vi "Log.vi"(8 "error in":errorcluster, 10 "Log Entry":T1 {"Time" format="%<%x %.3X>T"}, 11 "ILogger in":refnum<class "ILogger.lvclass">) -> (0 "error out":errorcluster, 3 "ILogger out":refnum<class "ILogger.lvclass">)   [LabVIEW 2026, in "ILogger.lvlib" / "ILogger.lvclass"]
doc: "Log the provided entry."
uses:
  ILogger.lvclass
  Type Definitions/Log Entry--cluster.ctl
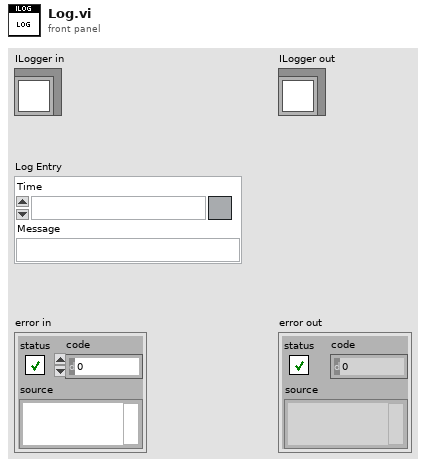
[diagram p1: front panel]
types:
  T1 = typedef "Log Entry--cluster.ctl" = cluster{"Time":timestamp, "Message":string}
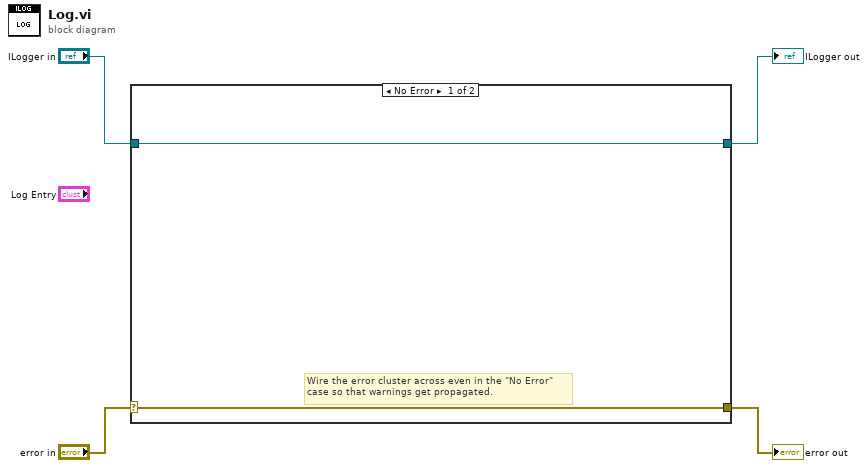
[diagram p0: block diagram]
diagram:
  n1 = case shown="No Error" "error in" {
    selector: "error in" -> [w6 w8]
    tunnel: [w6 w8] -> w3
    tunnel: [w5 w7] -> w1
    tunnel: "ILogger in" -> [w5 w7]
    frame No Error {
      # "Wire the error cluster across even in the \"No Error\"\ncase so that warnings get propagated."
    }
    frame Error {
    }
  }
  "error out" <- w3
  "ILogger out" <- w1
